vi "GAP_AcquireImagesV2_1.vi"() -> ()   [LabVIEW 2020]
uses:
  <vilib>/vision/driver/IMAQdx.llb/IMAQdx Buffer Number Mode.ctl
  <vilib>/vision/driver/NI_Vision_Acquisition_Software.lvlib
  <vilib>/vision/NI_Vision_Development_Module.lvlib
  <resource>/objmgr/imaqdx.rc
  Control 2.ctl
panel:
  in  "Tab Control":T1(tab)
  in  "Camera Name":refnum<k21> caption="IMAQdx Session"
  out "Original Image":T2(plugin-control)
  out "Grayscale Image":T2(plugin-control)
  out "Acquired imgs":u32
  out "Frame rate":dbl
  in  "Overwrite Mode":u16(ring) items=["Get Oldest"=0, "Fail"=2, "Get Newest"=3]
  in  "Percent of Images Reserved by Driver":dbl=50.0
  out "ROI information":T3 {"Minimum grayscale value" format="%.2f"; "Std. dev. of pixels values [ % ]" format="%.2f"; "Mean value of pixels values" format="%.2f"; "Maximum grayscale value" format="%.2f"}
  out "Line Profile":cluster{"x0":sgl, "dx":sgl, "Pixels Line":sgl[]}(graph)
  in  "Stop Button":bool
  in  "Start acquisition":bool
  in  "Stop image acquisition":bool
  in  "Save image":T4
  in  "stop":bool
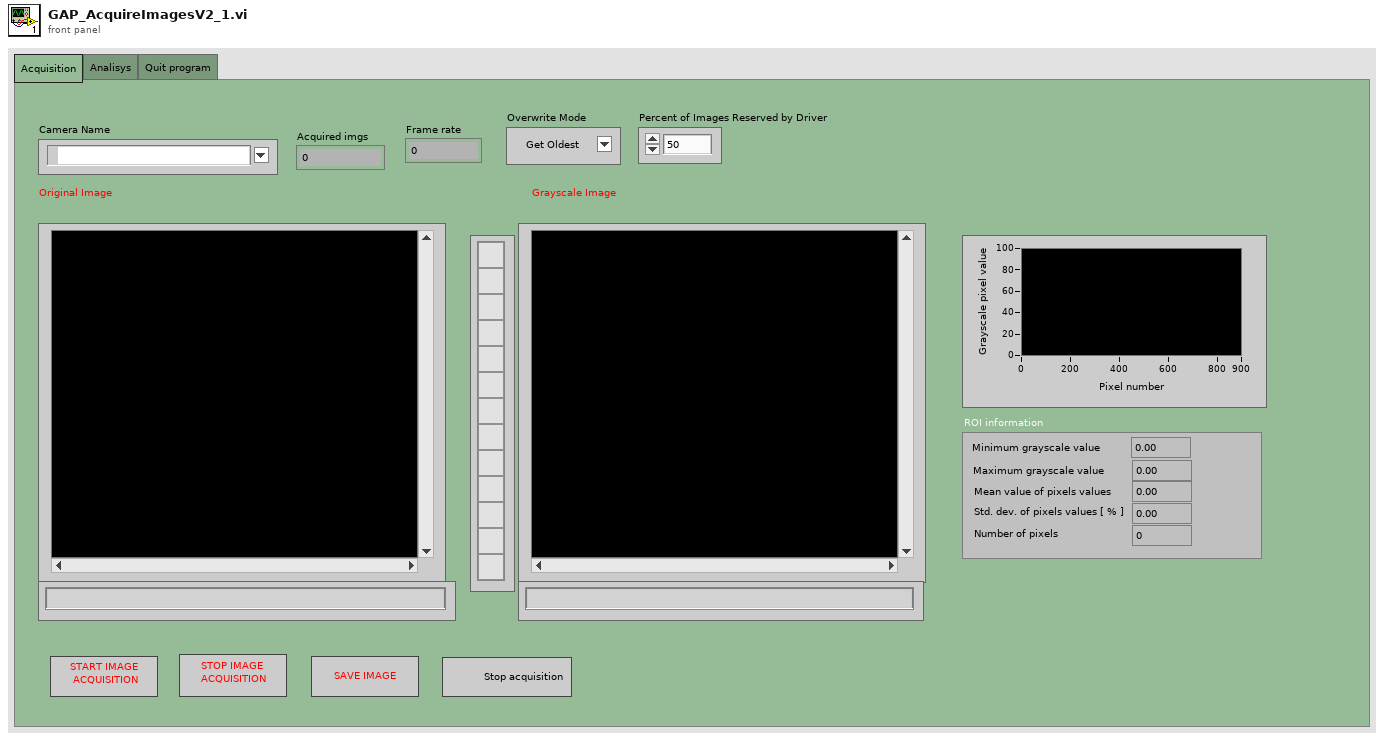
[diagram p1: front panel]
types:
  T1 = enum32{"Acquisition", "Analisys", "Quit program"}
  T2 = typedef "IMAQ Image.ctl" = refnum<image>
  T3 = cluster{"Minimum grayscale value":sgl, " Maximum grayscale value":sgl, "Mean value of pixels values":sgl, "Std. dev. of pixels values [ % ]":sgl, "Number of pixels":i32}
  T4 = typedef "Control 2.ctl" = bool
  T5 = typedef "NI_Vision_Acquisition_Software.lvlib/IMAQdx Buffer Number Mode.ctl" = enum32{"Next", "Last", "Buffer Number", "Every", "Last New"}
  T6 = typedef "Image Type" = u32
  T7 = typedef "IMAQdx.ctl" = refnum<k21>
  T8 = cluster{"Min":sgl, "Max":sgl, "Mean":sgl, "Std Dev":sgl, "Count":i32}
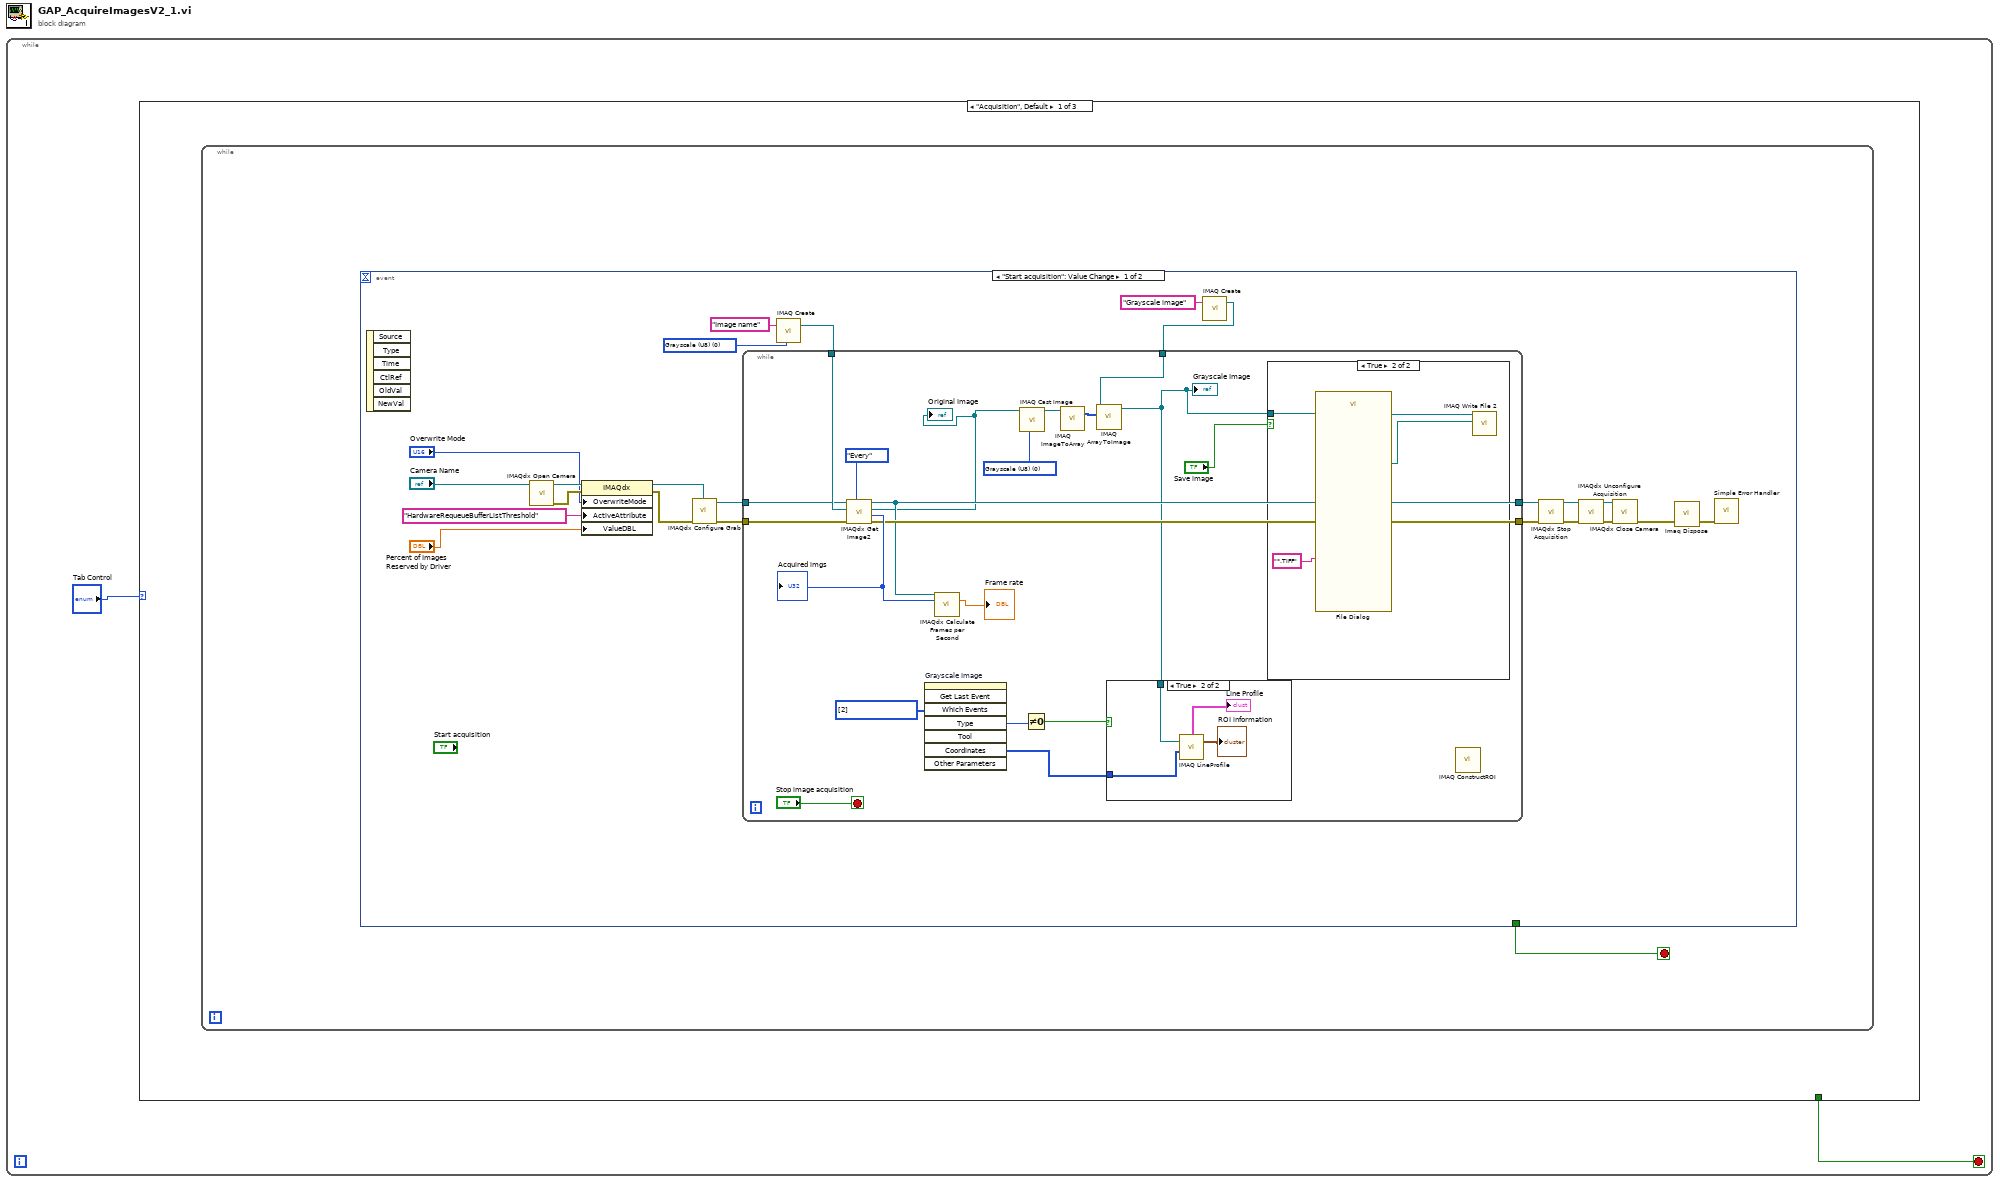
[diagram p0: block diagram]
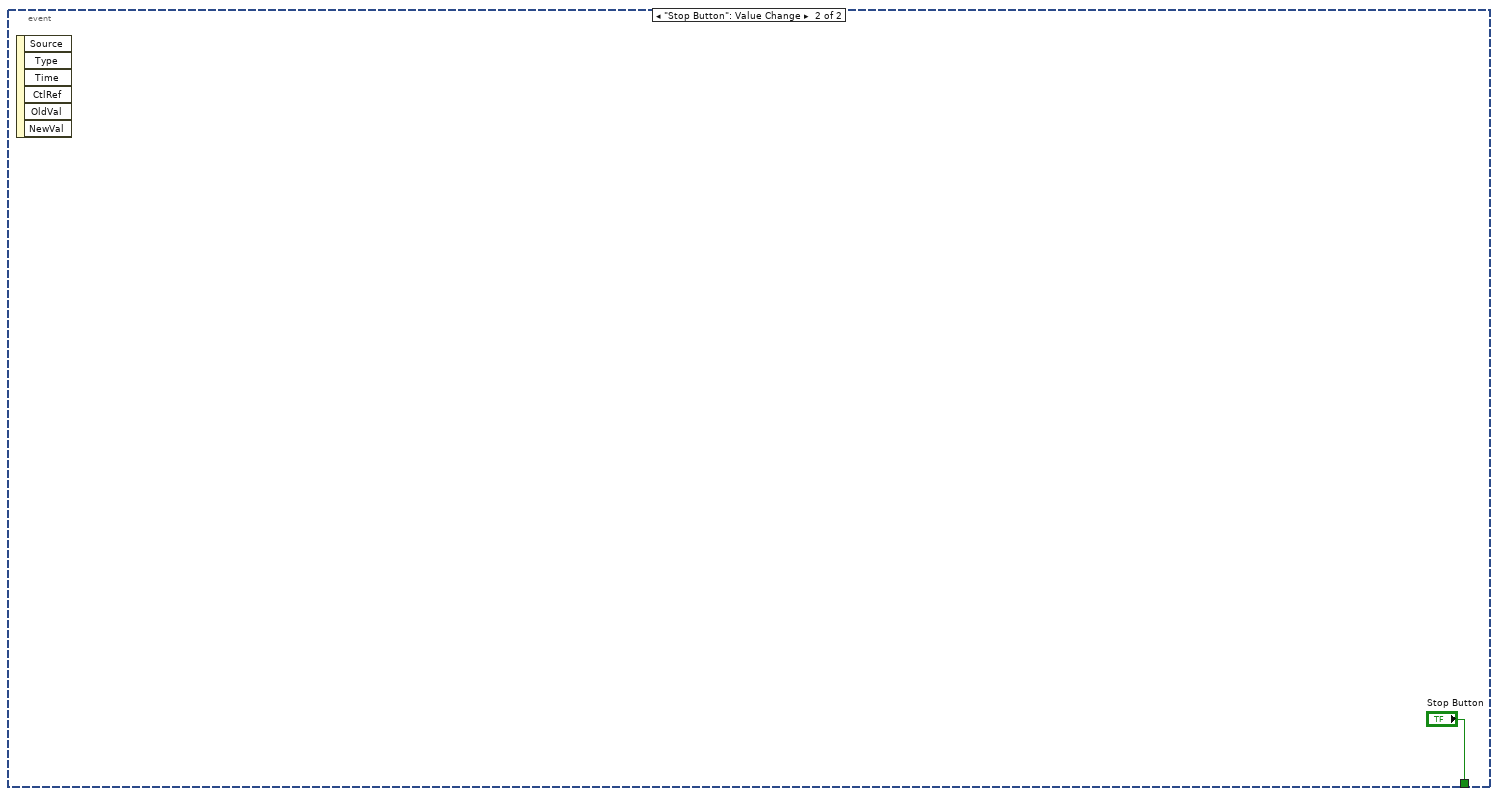
[diagram p4: hidden frame]
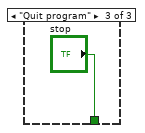
[diagram p6: hidden frame]
diagram:
  n1 = while {
    stop <- w1 stop-if-true
    n2 = case shown="\"Acquisition\", Default" "Tab Control" {
      tunnel: [_ _ "stop"] -> w1
      frame "Acquisition", Default {
        n3 = while {
          stop <- w3 stop-if-true
          n4 = event shown="[0] \"Start acquisition\": Value Change" {
            selector: _ -> [_ _]
            dyn-events: _ -> [_ _]
            timeout: _ -> [_ _]
            tunnel: [_ "Stop Button"] -> w3
            event "Start acquisition": Value Change {
              w4 = T6 0 items=["Grayscale (U8)", "Grayscale (I16)", "Grayscale (SGL)", "Complex (CSG)", "RGB (U32)", "HSL (U32)", "RGB (U64)", "Grayscale (U16)"] ("Image Type")
              n5 = event-data() -> ()  [unwired: 1 in, 6 out]
              n6 = call <vilib>:"IMAQdx Open Camera.vi"("Session In"="Camera Name") -> ("error out"=w23:errorcluster, "Session Out"=w24:T7)  [unwired: 2 in, 7 out]
              n7 = property class="IMAQdx"(reference=w24, error in=w23, "OverwriteMode"="Overwrite Mode", "ActiveAttribute"="HardwareRequeueBufferListThreshold", "ValueDBL"="Percent of Images Reserved by Driver") -> (reference out=w19:T7, error out=w20:errorcluster)
              n8 = call <vilib>:"IMAQdx Configure Grab.vi"("error in"=w20, "Session In"=w19) -> ("error out"=w17:errorcluster, "Session Out"=w18:T7)  [unwired: 8 in]
              n9 = call "IMAQ Create"("Image Name"="Image name", "Image Type"=w4) -> ("New Image"=w15:T2)  [unwired: 2 in, 2 out]
              n10 = call "IMAQ Create"("Image Name"="Grayscale image") -> ("New Image"=w5:T2)  [unwired: 3 in, 2 out]
              n11 = while {
                tunnel: w15 -> [w45]
                tunnel: w18 -> [w43]
                tunnel: w17 -> [w42]
                tunnel: [w41] -> w8
                tunnel: [w40] -> w7
                tunnel: w5 -> [w30]
                stop <- "Stop image acquisition" stop-if-true
                w33 = T6 0 items=["Grayscale (U8)", "Grayscale (I16)", "Grayscale (SGL)", "Complex (CSG)", "RGB (U32)", "HSL (U32)", "RGB (U64)", "Grayscale (U16)"] ("Image Type")
                w39 = i32[] [2] items=["No Event"=0, "Click Event"=1, "Draw Event"=2, "Size Event"=4, "Scroll Event"=5, "Double Click Event"=8] ("Which Events")
                n12 = call <vilib>:"IMAQdx Get Image2.vi"("Buffer Number Mode (Next)"=IMAQdx_Buffer_Number_Mode."Every", "error in"=w42, "Image In"=w45, "Session In"=w43) -> ("error out"=w41:errorcluster, "Buffer Number Out"=w46:u32, "Image Out"=w29:T2, "Session Out"=w40:T7)  [unwired: 4 in]
                "Acquired imgs" <- w46
                "Original Image" <- w29
                n13 = invoke on="Grayscale Image" class="ImageControl" method="Get Last Event"("Which Events"=w39) -> ("Type"=w38:i32, "Coordinates"=w36:i32[])  [unwired: 7 in, 6 out]
                n14 = call <vilib>:"IMAQdx Calculate Frames per Second.vi"("Session In"=w40, "Buffer Number"=w46) -> ("Acquired Frames per Second"=→"Frame rate":dbl)  [unwired: 7 in, 6 out]
                n15 = call "IMAQ Cast Image"("Image Type"=w33, "Image Src"=w29) -> ("Image Dst Out"=w32:T2)  [unwired: 4 in, 5 out]
                n16 = Not Equal To 0?(x=w38) -> (x != 0?=w37:bool)
                n17 = call "IMAQ ImageToArray"("Image"=w32) -> ("Image Pixels (U8)"=w31:u8[][])  [unwired: 3 in, 4 out]
                n18 = call "IMAQ ArrayToImage"("Image Pixels (U8)"=w31, "Image"=w30) -> ("Image Out"=w27:T2)  [unwired: 8 in, 1 out]
                "Grayscale Image" <- w27
                n19 = case shown="True" w37 {
                  tunnel: w36 -> [_ w52]
                  tunnel: w27 -> [_ w51]
                  frame False {
                  }
                  frame True {
                    n20 = call "IMAQ LineProfile"("Line Coordinates"=w52, "Image"=w51) -> ("Line Graph"=→"Line Profile":cluster{"x0":sgl, "dx":sgl, "Pixels Line":sgl[]}, "Line Information"=→"ROI information":T8)  [unwired: 3 in, 2 out]
                  }
                }
                n21 = case shown="True" "Save image" {
                  tunnel: w27 -> [_ w49]
                  frame False {
                  }
                  frame True {
                    n22 = call "File Dialog"("pattern (all files)"="*.TIFF" ("pattern label")) -> ("selected path"=w48:path)  [unwired: 11 in, 3 out]
                    n23 = call-poly "IMAQ Write File 2"("File Path"=w48, "Image"=w49) -> ()  [unwired: 8 in, 2 out]
                  }
                }
                n24 = call "IMAQ ConstructROI"() -> ()  [unwired: 8 in, 4 out]
              }
              n25 = call <vilib>:"IMAQdx Stop Acquisition.vi"("error in"=w8, "Session In"=w7) -> ("error out"=w10:errorcluster, "Session Out"=w11:T7)  [unwired: 8 out]
              n26 = call <vilib>:"IMAQdx Unconfigure Acquisition.vi"("error in"=w10, "Session In"=w11) -> ("error out"=w12:errorcluster, "Session Out"=w13:T7)  [unwired: 8 out]
              n27 = call <vilib>:"IMAQdx Close Camera.vi"("error in"=w12, "Session In"=w13) -> ("error out"=w9:errorcluster)  [unwired: 9 out]
              n28 = call "Imaq Dispose"("error in (no error)"=w9) -> ("error out"=w14:errorcluster)  [unwired: 5 in]
              n29 = call <vilib>:"Simple Error Handler.vi"("error in (no error)"=w14) -> ()  [unwired: 4 in, 5 out]
            }
            event "Stop Button": Value Change {
              n30 = event-data() -> ()  [unwired: 1 in, 6 out]
            }
          }
        }
      }
      frame "Analisys" {
      }
      frame "Quit program" {
      }
    }
  }
